vi "ejemplo-de-procesado-de-senales.vi"() -> ()   [LabVIEW 2019]
uses:
  <vilib>/express/express analysis/Spectral/Block/exnSpectralBlock spectral measurements PSD poly.vi
  <vilib>/express/express analysis/Spectral/Block/exnSpectralBlock spectral measurements PSD WFM.vi
  <vilib>/express/express analysis/Spectral/Block/exnSpectralBlock spectral measurements PSD DDT.vi
  <vilib>/express/express analysis/Spectral/XNode/ExpressSpectralMeasurementsBlockNode.xnode
  <vilib>/measure/NI_MAPro.lvlib
panel:
  out "Waveform Graph 3":dynamicdata(graph)
  out "Filtered Signal":dynamicdata(graph)
  out "Waveform Graph 2":cluster{"f0":dbl, "df":dbl, "magnitude":dbl[]}(graph)
  out "Waveform Graph":waveform(dbl)(graph)
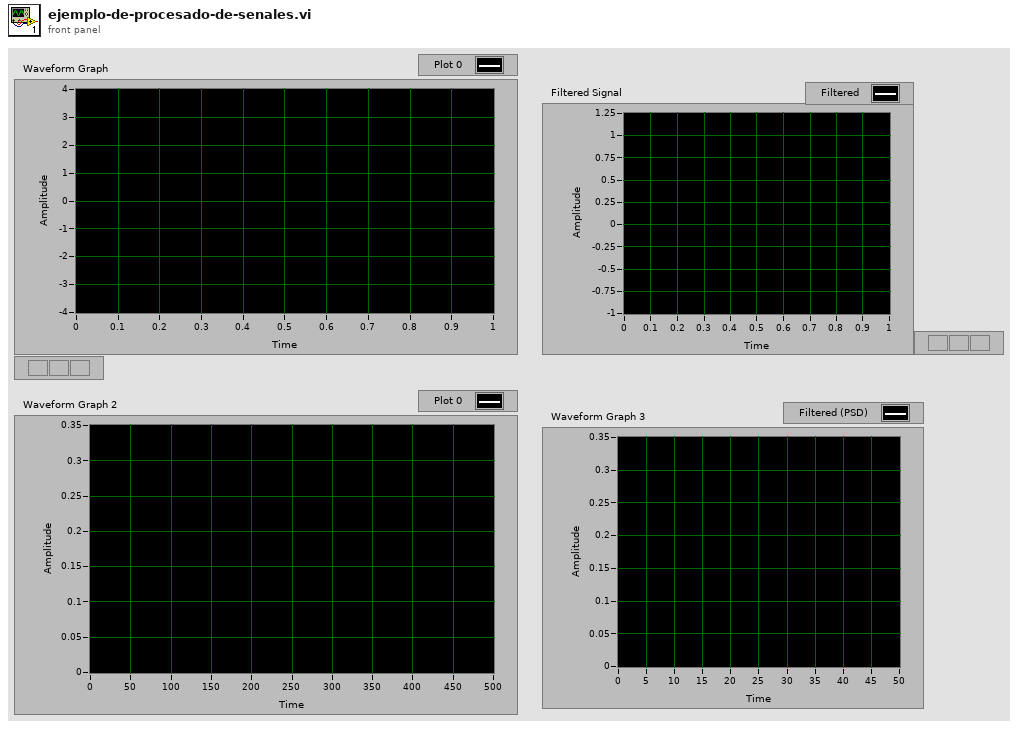
[diagram p1: front panel]
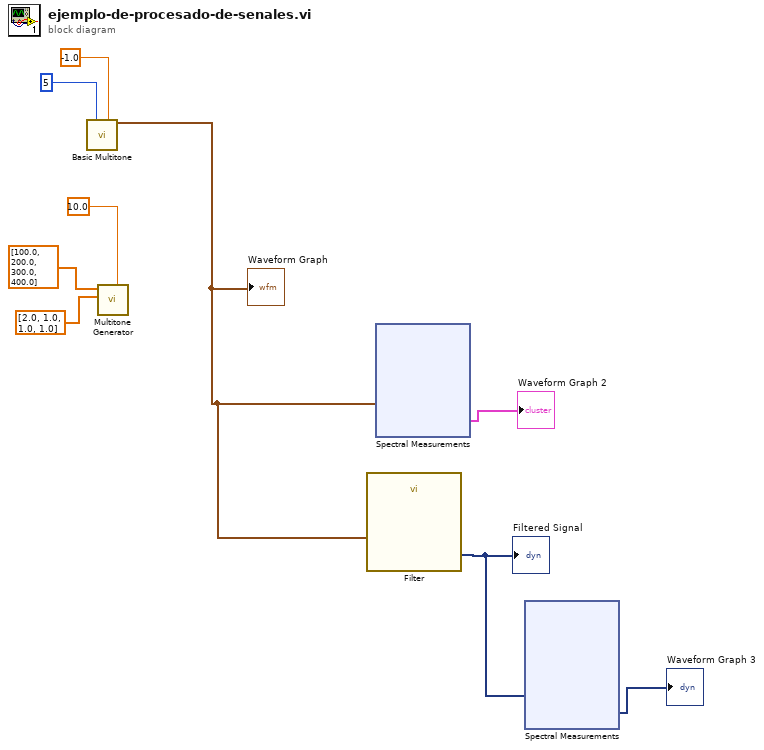
[diagram p0: block diagram]
diagram:
  n1 = call <vilib>:"Basic Multitone.vi"("#tones"=5, "amplitude"=-1.0) -> ("signal out"=w1:waveform(dbl))  [unwired: 10 in, 3 out]
  "Waveform Graph" <- w1
  n2 = call <vilib>:"Multitone Generator.vi"("amplitude"=10.0, "tone amplitudes"=dbl[] [2.0, 1.0, 1.0, 1.0], "tone frequencies"=dbl[] [100.0, 200.0, 300.0, 400.0]) -> ()  [unwired: 5 in, 4 out]
  n3 = call "Filter"("Signal"=w1) -> ("Filtered Signal"=w5:dynamicdata)  [unwired: 9 in, 1 out]
  "Filtered Signal" <- w5
  n4 = xnode "Spectral Measurements"("Signals"=w1) -> ("PSD"=→"Waveform Graph 2":cluster{"f0":dbl, "df":dbl, "magnitude":dbl[]})  [unwired: 1 in, 1 out]
  n5 = xnode "Spectral Measurements"("Signals"=w5) -> ("PSD"=→"Waveform Graph 3":dynamicdata)  [unwired: 1 in, 1 out]
